vi "Add CTRLs By VI Reference.vi"(8 "error in (no error)":errorcluster, 11 "VIs in":refnum<vi>[](array[refnum])) -> (0 "error out":errorcluster, 3 "VIs out":refnum<vi>[](array[refnum]))   [LabVIEW 2019, in "Language Selection.lvlib"]
doc: "Add additional controls to translate selection by VI references.\n- - -\nCopyright (c) 2026, Merecs Engineering GmbH"
uses:
  Language Selection.lvlib
panel:
  # "Connector Pane"
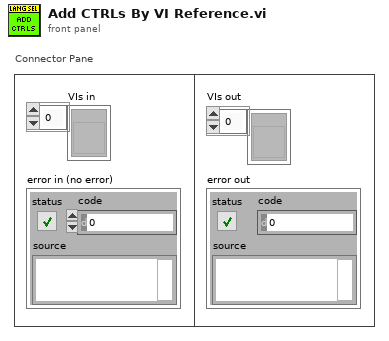
[diagram p1: front panel]
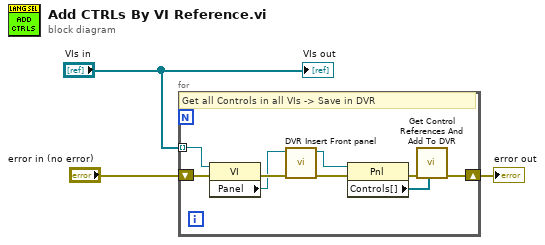
[diagram p0: block diagram]
diagram:
  n1 = for {
    tunnel: "VIs in" -> [w11] mode=indexing
    shift-right: [w4] -> w2
    shift-left: "error in (no error)" -> [w12]
    # "Get all Controls in all VIs -> Save in DVR"
    n2 = property class="VI"(reference=w11, error in=w12) -> (error out=w8:errorcluster, "Panel"=w6:refnum<vi>)  [unwired: 1 out]
    n3 = call "DVR Insert Front panel.vi"("error in (no error)"=w8, "Panel in"=w6) -> ("error out"=w7:errorcluster, "Panel out"=w5:refnum<vi>)  [unwired: 8 in]
    n4 = property class="Pnl"(reference=w5, error in=w7) -> (error out=w9:errorcluster, "Controls[]"=w10:refnum<vi>[])  [unwired: 1 out]
    n5 = call "Get Control References And Add To DVR.vi"("Controls[]"=w10, "error in (no error)"=w9) -> ("error out"=w4:errorcluster)  [unwired: 9 in]
  }
  "error out" <- w2
  "VIs out" <- "VIs in"
